vi "configure operation.vi"(7 "owner ID":refnum<class "Profibus Module configuration.lvclass">, 8 "error in":errorcluster, 10 "line item in":T1, 11 "engine configuration in":refnum<class "engine configuration.lvclass">) -> (0 "error out":errorcluster, 1 "success":bool, 2 "line item out":T1, 5 "changed":bool)   [LabVIEW 2013, in "Profibus Module editor node.lvclass"]
uses:
  Profibus Module editor node.lvclass
  permissions.ctl
  table line.ctl
  channel/Profibus channel.lvclass
  <vilib>/NI/Module Execution Interface/Engine Configuration/engine configuration.lvclass
  configuration/Profibus Module configuration.lvclass
  <vilib>/NI/Configuration Framework/serializable configuration/NISE_CEF_serializable configuration.lvclass/NISE_CEF_serializable configuration.ctl
  <vilib>/NI/Tag Bus Module Framework/channel/TBM channel.lvclass/TBM channel.ctl
  <vilib>/NI/Tag Bus/tag/tag descriptor.lvclass/tag descriptor.ctl
  channel/Profibus channel.lvclass/Profibus channel.ctl
  <vilib>/NI/Tag Bus/tag/Data Type.ctl
  <vilib>/NI/Configuration Framework/serializable configuration/Read UID.vi
  <vilib>/NI/Tag Bus Module Framework/channel/Read channel classification.vi
  <vilib>/NI/Tag Bus/tag/read data type.vi
  channel/Read slave.vi
  channel/Read byte.vi
  channel/Read bit.vi
  <vilib>/NI/Tag Bus/tag/write tag name.vi
  <vilib>/NI/Tag Bus/tag/write data type.vi
  <vilib>/NI/Tag Bus Module Framework/channel/Write channel classification.vi
  channel/Write slave.vi
  channel/Write byte.vi
  channel/Write bit.vi
  <vilib>/Utility/LVClass/Get LV Class Name.vi
  <vilib>/NI/Configuration Framework/error generator/NISE_error generator.vi
  <vilib>/NI/Tag Bus/tag/tag descriptor.lvclass
panel:
  in  "Linked Tag":i32(listbox)
  in  "Data Type":i32(listbox)
  in  "bit":i32
  in  "byte":i32
  in  "slave":i8
  in  "Channel Name":string
  in  "cancel":bool
  in  "ok":bool
  in  "Access Type":T2
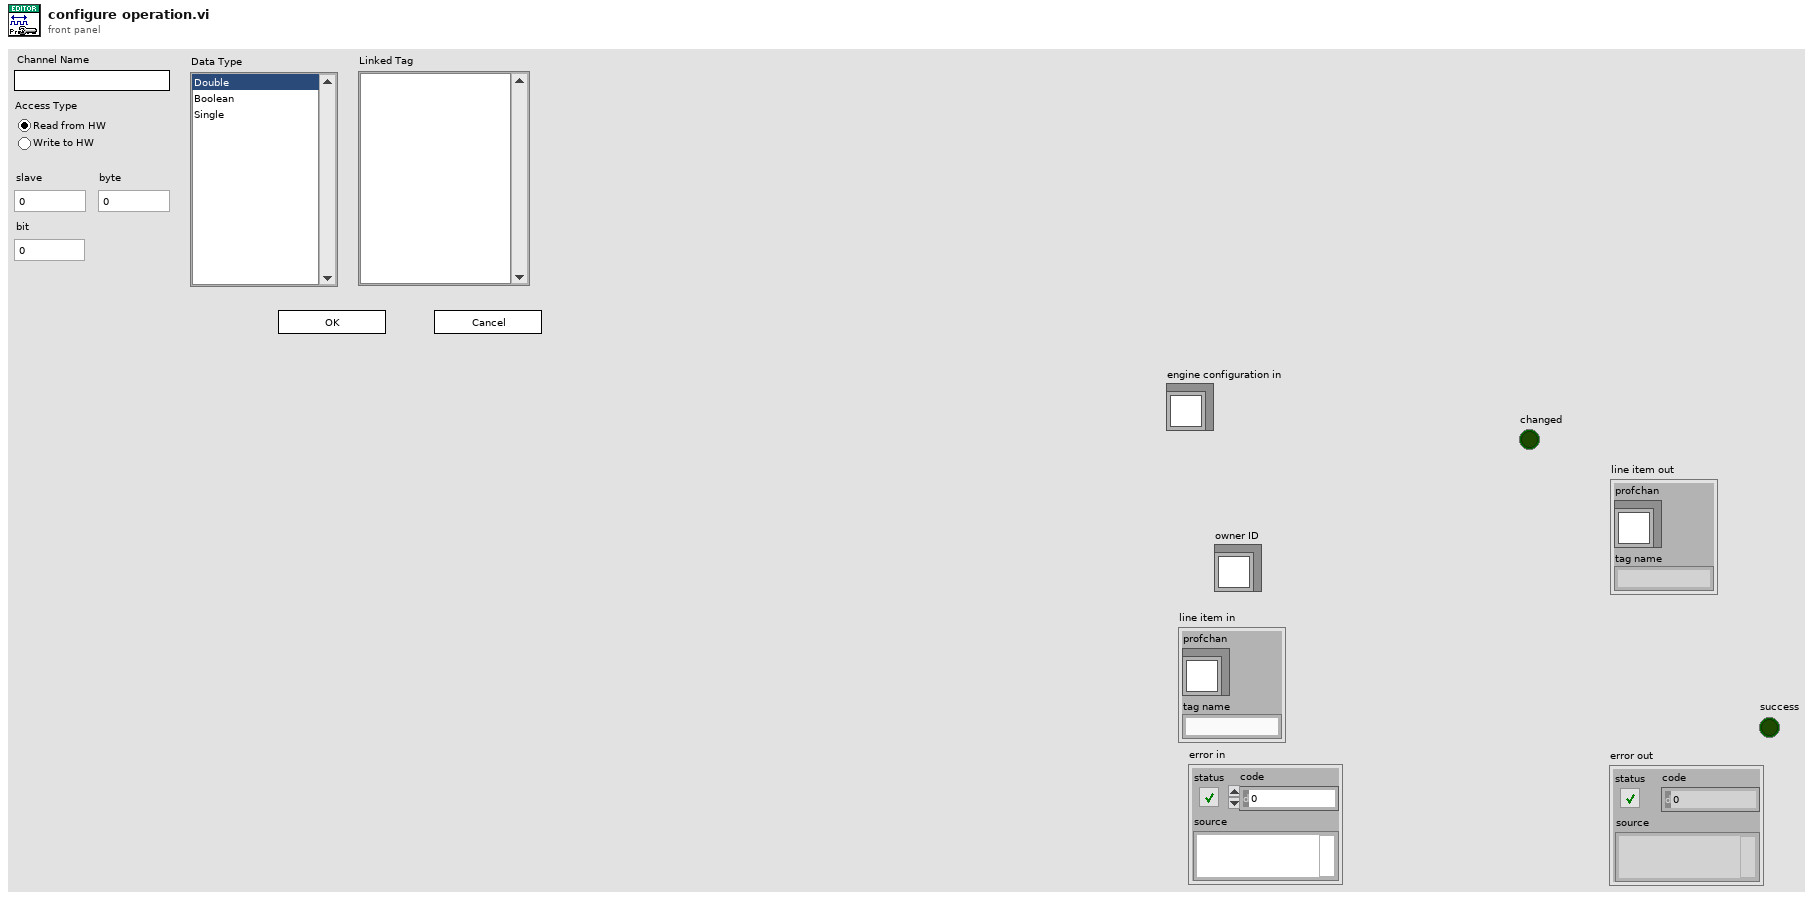
[diagram p1: front panel]
types:
  T1 = typedef "Profibus Module editor node.lvclass/table line.ctl" = cluster{"profchan":refnum<class "Profibus channel.lvclass">, "tag name":string}
  T2 = typedef "Profibus Module editor node.lvclass/permissions.ctl" = enum32{"Read from HW", "Write to HW"}
  T3 = enum32{"Invalid", "Standard", "Closed", "Hidden", "Minimized", "Maximized"}
  T4 = enum32{"Invalid", "Default", "Floating", "Floating/Auto-Hide", "Modal"}
  T5 = enum8{"Enabled", "Disabled", "Disabled and Grayed Out"}
  T6 = typedef "tag bus.lvlib/tag descriptor.lvclass/Data Type.ctl" = enum16{"Double", "Single", "I64", "I32", "I16", "I8", "U64", "U32", "U16", "U8", "Boolean", "String", "Array of Double", "Array of Single", "Array of I64", "Array of I32", "Array of I16", "Array of I8", "Array of U64", "Array of U32", "Array of U16", "Array of U8", "Array of Boolean", "Array of String"}
  T7 = enum32{"invalid app kind", "Development System", "Run Time System", "Student Edition", "Embedded LabVIEW", "Evaluation", "Custom"}
  T8 = typedef "TBM channel.lvclass/channel classification.ctl" = enum16{"input data", "output data", "processing parameter", "processing result"}
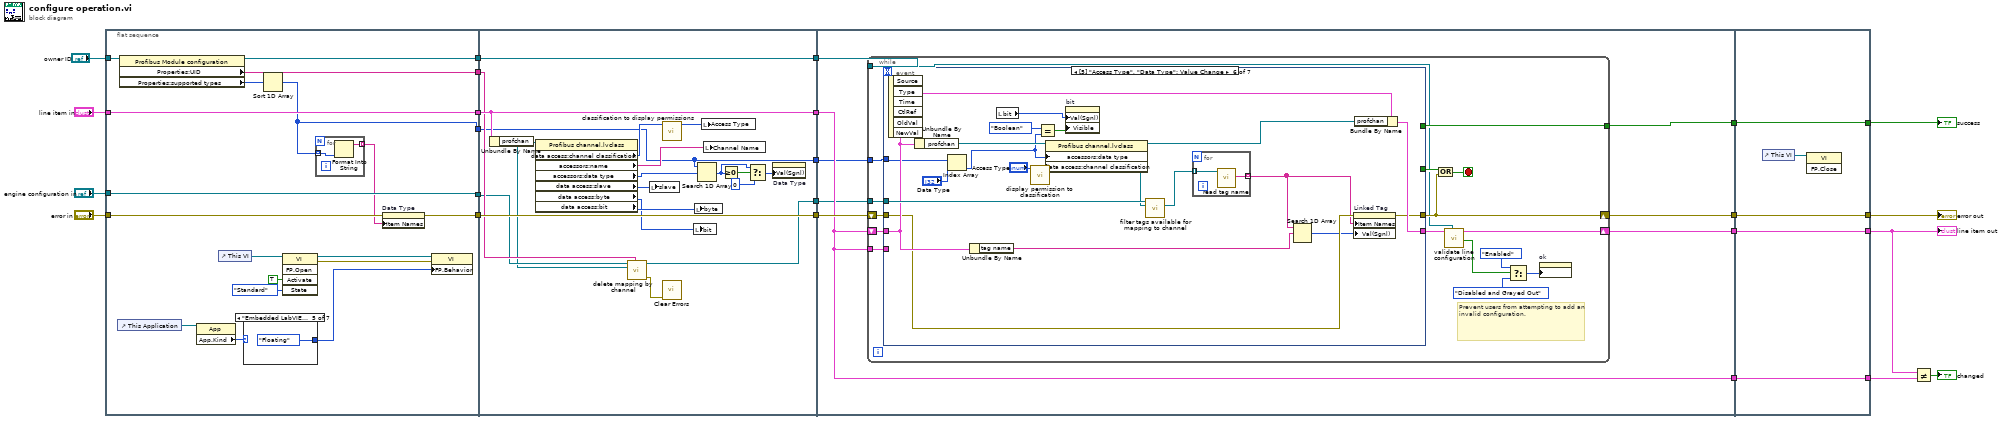
[diagram p0: block diagram]
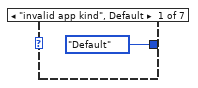
[diagram p2: hidden frame]
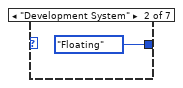
[diagram p3: hidden frame]
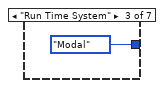
[diagram p4: hidden frame]
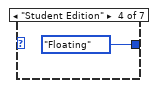
[diagram p5: hidden frame]
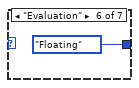
[diagram p6: hidden frame]
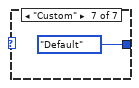
[diagram p7: hidden frame]
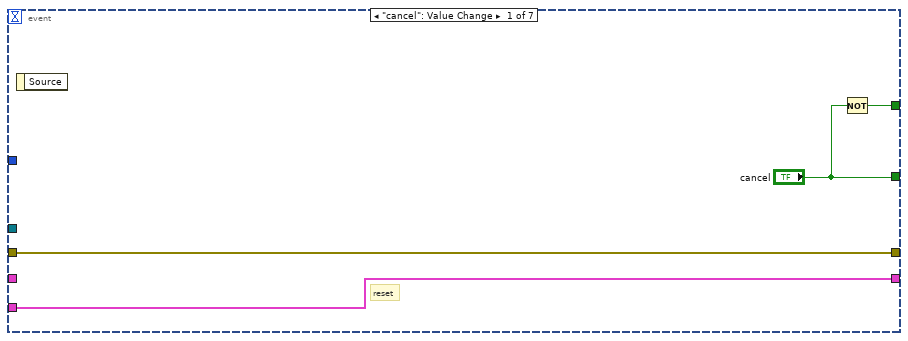
[diagram p8: hidden frame]
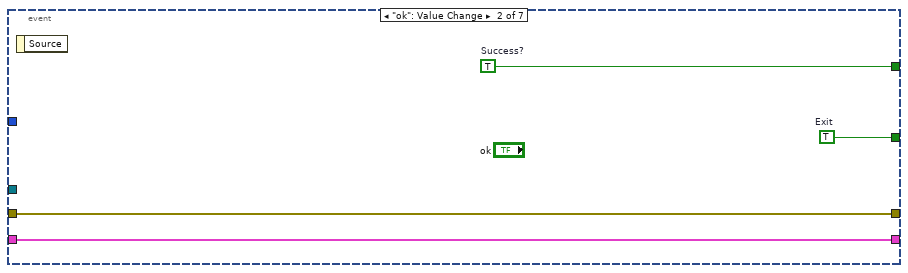
[diagram p9: hidden frame]
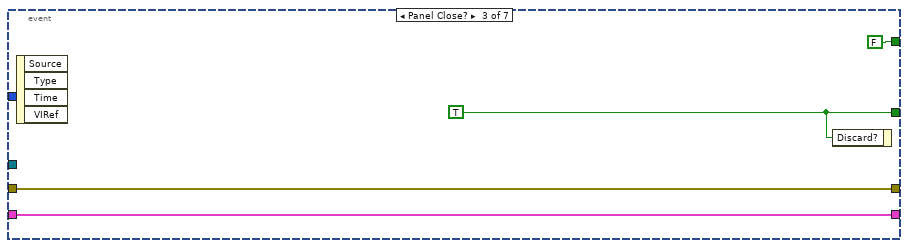
[diagram p10: hidden frame]
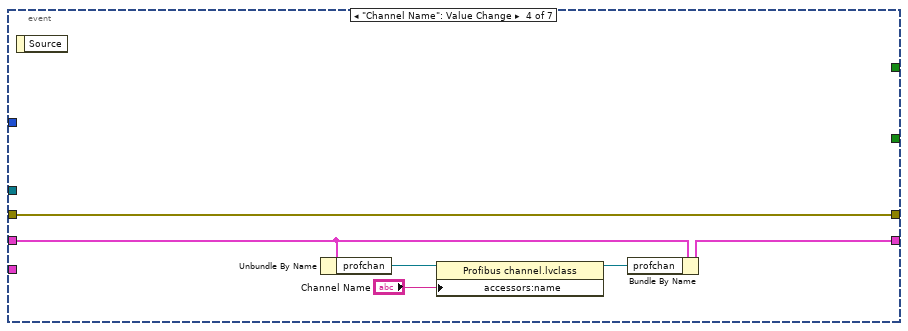
[diagram p11: hidden frame]
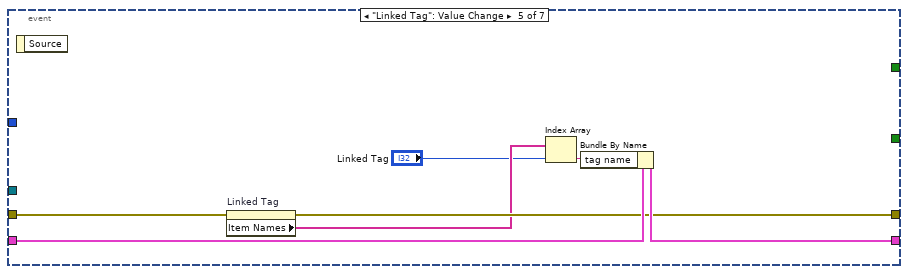
[diagram p12: hidden frame]
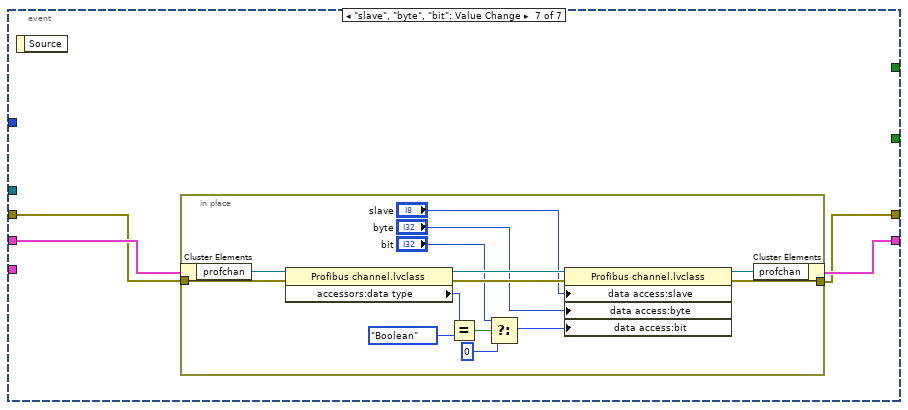
[diagram p13: hidden frame]
diagram:
  n1 = flat-sequence {
    tunnel: "line item in" -> [w42]
    tunnel: "error in" -> [w29]
    tunnel: [w28] -> w13
    tunnel: [w42] -> w11
    tunnel: [w31] -> w8
    tunnel: "owner ID" -> [w33]
    tunnel: [w32] -> w6
    tunnel: "engine configuration in" -> [w32]
    tunnel: [w30] -> w3
    tunnel: [w25] -> w2
    tunnel: w13 -> [w71]
    tunnel: [w71] -> w12
    tunnel: w11 -> [w67]
    tunnel: [w67] -> w10
    tunnel: [w63] -> w9
    tunnel: w8 -> [w63]
    tunnel: w6 -> [w60]
    tunnel: [w62] -> w4
    tunnel: w3 -> [w61]
    tunnel: w2 -> [w53]
    tunnel: [w53] -> w1
    tunnel: [w78] -> w17
    tunnel: [w77] -> w16
    tunnel: [w76] -> w15
    tunnel: [w75] -> w14
    tunnel: w12 -> [w79]
    tunnel: w10 -> [w75]
    tunnel: w9 -> [w74]
    tunnel: w4 -> [w73]
    tunnel: w1 -> [w72]
    tunnel: [w161] -> w18
    tunnel: [w162] -> w21
    tunnel: [w163] -> w22
    tunnel: [w164] -> w23
    tunnel: w17 -> [w164]
    tunnel: w16 -> [w163]
    tunnel: w15 -> [w162]
    tunnel: w14 -> [w161]
    frame #0 {
      n2 = control-ref of="This Application"() -> (w36:refnum<vi>)
      n3 = property class="Profibus Module configuration"(reference=w33) -> (reference out=w31:refnum<class "Profibus Module configuration.lvclass">, "Properties:UID"=w30:string, "Properties:supported types"=w26:T6[])  [unwired: 1 in, 1 out]
      n4 = property class="App"(reference=w36) -> ("App.Kind"=w35:T7)  [unwired: 1 in, 2 out]
      n5 = control-ref of="This VI"() -> (w37:refnum<vi>)
      n6 = case shown="\"Embedded LabVIEW\"" w35 {
        tunnel: [T4."Default" ("Front Panel Window:Behavior") T4."Floating" ("Front Panel Window:Behavior") T4."Modal" ("Front Panel Window:Behavior") T4."Floating" ("Front Panel Window:Behavior") T4."Floating" ("Front Panel Window:Behavior") T4."Floating" ("Front Panel Window:Behavior") T4."Default" ("Front Panel Window:Behavior")] -> w34
        frame "invalid app kind", Default {
        }
        frame "Development System" {
        }
        frame "Run Time System" {
        }
        frame "Student Edition" {
        }
        frame "Embedded LabVIEW" {
        }
        frame "Evaluation" {
        }
        frame "Custom" {
        }
      }
      n7 = Sort 1D Array(array=w26) -> (sorted array=w25:T6[])
      n8 = invoke class="VI" method="FP.Open"(reference=w37, "Activate"=TRUE ("Activate?"), "State"=T3."Standard") -> (reference out=w40:refnum<vi>, error out=w41:errorcluster)  [unwired: 2 in, 3 out]
      n9 = for {
        tunnel: w25 -> [w44] mode=indexing
        tunnel: [w43] -> w27 mode=indexing
        n10 = Format Into String(w44) -> (resulting string=w43:string)  [unwired: 3 in, 1 out]
      }
      n11 = property on="Data Type" class="LstBox (strict)"(error in=w29, "Item Names"=w27) -> (error out=w28:errorcluster)  [unwired: 1 in, 1 out]
      n12 = property class="VI"(reference=w40, error in=w41, "FP.Behavior"=w34) -> ()  [unwired: 2 out]
    }
    frame #1 {
      n13 = Unbundle By Name(w67) -> ("profchan"=w59:refnum<class "Profibus channel.lvclass">)
      n14 = property class="Profibus channel.lvclass"(reference=w59) -> ("data access:channel classification"=w70:T8, "accessors:name"=w69:string, "accessors:data type"=w57:T6, "data access:slave"=w64:i8, "data access:byte"=w66:i32, "data access:bit"=w65:i32)  [unwired: 1 in, 2 out]
      n15 = call <vilib>:"delete mapping by channel.vi"("owner ID"=w61, "channel"=w59, "engine configuration in"=w60) -> ("error out"=w58:errorcluster, "engine configuration out"=w62:refnum<class "engine configuration.lvclass">)  [unwired: 7 in]
      n16 = local write "slave"(w64) -> ()
      n17 = call "classification to display permissions.vi"("channel classification"=w70) -> ("permissions"=w68:T2)  [unwired: 10 in]
      n18 = call <vilib>:"Clear Errors.vi"("error in (no error)"=w58) -> ()  [unwired: 6 in, 1 out]
      n19 = local write "bit"(w65) -> ()
      n20 = local write "byte"(w66) -> ()
      n21 = Search 1D Array(1D array=w53, element=w57) -> (index of element=w55:i32)  [unwired: 1 in]
      n22 = local write "Access Type"(w68) -> ()
      n23 = local write "Channel Name"(w69) -> ()
      n24 = Greater Or Equal To 0?(x=w55) -> (x >= 0?=w56:bool)
      n25 = Select(t=w55, s=w56, f=0) -> (s? t:f=w52:i32)
      n26 = property on="Data Type" class="LstBox (strict)"("Val(Sgnl)"=w52) -> ()  [unwired: 2 in, 2 out]
    }
    frame #2 {
      n27 = while {
        shift-right: [w87] -> w77
        shift-left: w79 -> [w82]
        tunnel: [w94] -> w78
        shift-right: [w88] -> w76
        shift-left: w75 -> [w91]
        tunnel: w75 -> [w90]
        tunnel: w74 -> [w81]
        tunnel: w72 -> [w80]
        tunnel: w73 -> [w95]
        stop <- w92 stop-if-true
        # "Prevent users from attempting to add an invalid configuration."
        n28 = event shown="[5] \"Access Type\", \"Data Type\": Value Change" {
          selector: _ -> [_ _ _ _ _ _ _]
          dyn-events: _ -> [_ _ _ _ _ _ _]
          timeout: _ -> [_ _ _ _ _ _ _]
          tunnel: w95 -> [_ _ _ _ _ w137 _]
          tunnel: w82 -> [w99 w103 w107 w113 w117 w124 w142]
          tunnel: [w99 w103 w107 w113 w116 w125 w143] -> w87
          tunnel: [w98 w100 FALSE _ _ _ _] -> w94
          tunnel: ["cancel" w101 w105 _ _ _ _] -> w93
          tunnel: w91 -> [_ w102 w104 w111 w120 w135 w145]
          tunnel: [w96 w102 w104 w112 w119 w129 w144] -> w89
          tunnel: w90 -> [w96 _ _ _ _ _ _]
          tunnel: w80 -> [_ _ _ _ _ w128 _]
          event "cancel": Value Change {
            # "reset"
            n29 = event-data() -> ()  [unwired: 1 in, 1 out]
            n30 = Not(x="cancel") -> (.not. x?=w98:bool)
          }
          event "ok": Value Change {
            w100 = TRUE  # Success?
            w101 = TRUE  # Exit
            n31 = event-data() -> ()  [unwired: 1 in, 1 out]
          }
          event Panel Close? {
            w105 = TRUE ("cancel")
            n32 = event-data() -> ()  [unwired: 1 in, 4 out]
            n33 = event-data("Discard?"=w105) -> ()  [unwired: 1 in, 1 out]
          }
          event "Channel Name": Value Change {
            n34 = event-data() -> ()  [unwired: 1 in, 1 out]
            n35 = Unbundle By Name(w111) -> ("profchan"=w110:refnum<class "Profibus channel.lvclass">)
            n36 = property class="Profibus channel.lvclass"(reference=w110, "accessors:name"="Channel Name") -> (reference out=w109:refnum<class "Profibus channel.lvclass">)  [unwired: 1 in, 1 out]
            n37 = Bundle By Name(cluster=w111, "profchan"=w109) -> (w112:T1)
          }
          event "Linked Tag": Value Change {
            n38 = event-data() -> ()  [unwired: 1 in, 1 out]
            n39 = property on="Linked Tag" class="LstBox (strict)"(error in=w117) -> (error out=w116:errorcluster, "Item Names"=w115:string[])  [unwired: 1 in, 1 out]
            n40 = Index Array(array=w115, index="Linked Tag") -> (element=w118:string)
            n41 = Bundle By Name(cluster=w120, "tag name"=w118) -> (w119:T1)
          }
          event "Data Type": Value Change {
            n42 = event-data() -> ()  [unwired: 1 in, 6 out]
            n43 = Unbundle By Name(w135) -> ("profchan"=w130:refnum<class "Profibus channel.lvclass">)
            n44 = Index Array(array=w128, index="Data Type") -> (element=w126:T6)
            n45 = Unbundle By Name(w135) -> ("tag name"=w122:string)
            n46 = local read "bit"() -> (w131:i32)
            n47 = call "display permission to classification.vi"("display permissions"="Access Type") -> ("channel classification"=w138:T8)  [unwired: 10 in]
            n48 = Equal?(x=Data_Type."Boolean", y=w126) -> (x = y?=w132:bool)
            n49 = property class="Profibus channel.lvclass"(reference=w130, "accessors:data type"=w126, "data access:channel classification"=w138) -> (reference out=w136:refnum<class "Profibus channel.lvclass">)  [unwired: 1 in, 1 out]
            n50 = property on="bit" class="DigNum (strict)"("Val(Sgnl)"=w131, "Visible"=w132) -> ()  [unwired: 2 in, 2 out]
            n51 = call <vilib>:"filter tags available for mapping to channel.vi"("channel to map to"=w136, "engine configuration in"=w137) -> ("filtered tags"=w134:refnum<class "tag descriptor.lvclass">[])  [unwired: 8 in, 1 out]
            n52 = for {
              tunnel: w134 -> [w141] mode=indexing
              tunnel: [w140] -> w123 mode=indexing
              n53 = call <vilib>:"read tag name.vi"("system tag in"=w141) -> ("name"=w140:string)  [unwired: 8 in, 2 out]
            }
            n54 = Search 1D Array(1D array=w123, element=w122) -> (index of element=w121:i32)  [unwired: 1 in]
            n55 = property on="Linked Tag" class="LstBox (strict)"(error in=w124, "Item Names"=w123, "Val(Sgnl)"=w121) -> (error out=w125:errorcluster)  [unwired: 1 in, 1 out]
            n56 = Bundle By Name(cluster=w135, "profchan"=w136) -> (w129:T1)
          }
          event "slave", "byte", "bit": Value Change {
            n57 = event-data() -> ()  [unwired: 1 in, 1 out]
            n58 = in-place {
              in-place-border: [w155] -> w143
              in-place-border: w142 -> [w154]
              n59 = in-place-cluster #1(w145) -> ("profchan"=w159:refnum<class "Profibus channel.lvclass">)
              n60 = property class="Profibus channel.lvclass"(reference=w159, error in=w154) -> (reference out=w157:refnum<class "Profibus channel.lvclass">, error out=w156:errorcluster, "accessors:data type"=w153:T6)
              n61 = Equal?(x=w153, y=Data_Type."Boolean") -> (x = y?=w151:bool)
              n62 = Select(t="bit", s=w151, f=0) -> (s? t:f=w148:i32)
              n63 = property class="Profibus channel.lvclass"(reference=w157, error in=w156, "data access:slave"="slave", "data access:byte"="byte", "data access:bit"=w148) -> (reference out=w158:refnum<class "Profibus channel.lvclass">, error out=w155:errorcluster)
              n64 = in-place-cluster #1("profchan"=w158) -> (w144:T1)
            }
          }
        }
        n65 = Compound Arithmetic op=OR(w93, w87) -> (w92:bool)
        n66 = call "validate line configuration.vi"("Profibus Module configuration"=w81, "line in"=w89) -> ("valid?"=w86:bool, "line out"=w88:T1)  [unwired: 8 in]
        n67 = Select(t=T5."Enabled" ("Disabled"), s=w86, f=T5."Disabled and Grayed Out") -> (s? t:f=w83:T5)
        n68 = property on="ok" class="Bool"("DisabledEnum"=w83) -> ()  [unwired: 2 in, 2 out]
      }
    }
    frame #3 {
      n69 = control-ref of="This VI"() -> (w160:refnum<vi>)
      n70 = invoke class="VI" method="FP.Close"(reference=w160) -> ()  [unwired: 2 in, 3 out]
    }
  }
  n71 = Not Equal?(x=w21, y=w18) -> (x != y?=→"changed":bool)
  "error out" <- w22
  "success" <- w23
  "line item out" <- w21
